vi "Assert Greater Or Equal_Variant.vi"(4 "Execution time (s)":dbl=-1.0, 5 "Assert Only? (F)":bool, 6 "error code (1)":i32=1, 7 "Label":string, 8 "error in (no error)":errorcluster, 9 "Register with caller test (F)":bool, 10 "Y":variant, 11 "X":variant) -> (0 "error out":errorcluster, 2 "Properties.Assert":refnum<class "Properties.Assert.lvclass">)   [LabVIEW 2020, in "Caraya.lvlib" / "Assert.lvclass"]
doc: "Generates an error if the input condition is not met.\n\n--\nCopyright © 2015 JKI All rights reserved.\n\nAuthor: Tomi Maila <tomi.maila@jki.net>\n\nThis library is provided \"AS IS\" ,WITHOUT WARRANTIES OR\nCONDITIONS OF ANY KIND, either express or implied.\n\nJKI -- jki.net"
uses:
  Assert.lvclass
  Assert.lvclass/Assert.ctl
  <userlib>/_OpenG.lib/string/string.llb/openg_string.lvlib
  Properties/Properties.lvclass
  Properties.Assert/Properties.Assert.lvclass
  C:/Projects/caraya/src/classes/Properties/Properties.lvclass
  C:/Projects/caraya/src/classes/Properties.Assert/Properties.Assert.lvclass
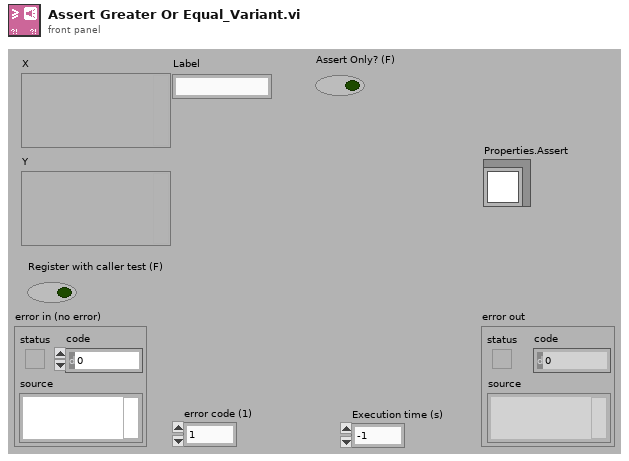
[diagram p1: front panel]
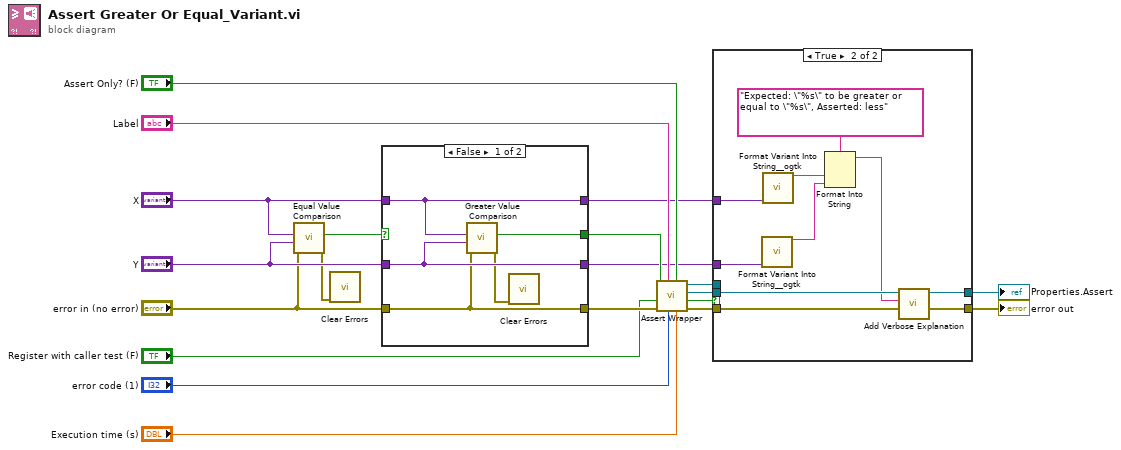
[diagram p0: block diagram]
diagram:
  n1 = call "Equal Value Comparison.vi"("error in (no error)"="error in (no error)", "Actual"="Y", "Expected"="X") -> ("error out"=w5:errorcluster, "Equal Values?"=w7:bool)  [unwired: 6 in, 1 out]
  n2 = call <vilib>:"Clear Errors.vi"("error in (no error)"=w5) -> ()  [unwired: 5 in, 2 out]
  n3 = case shown="False" w7 {
    selector: w7 -> [_ w28]
    tunnel: "X" -> [w25 w29]
    tunnel: [w25 w29] -> w13
    tunnel: [w23 w28] -> w12
    tunnel: "Y" -> [w24 w27]
    tunnel: [w24 w27] -> w11
    tunnel: "error in (no error)" -> [w22 w26]
    tunnel: [w22 w26] -> w10
    frame False {
      n4 = call "Greater Value Comparison.vi"("error in (no error)"=w22, "Y"=w24, "X"=w25) -> ("error out"=w21:errorcluster, "Asserted?"=w23:bool)  [unwired: 6 in, 1 out]
      n5 = call <vilib>:"Clear Errors.vi"("error in (no error)"=w21) -> ()  [unwired: 5 in, 2 out]
    }
    frame True {
    }
  }
  n6 = call "Assert Wrapper.vi"("Execution time (s)"="Execution time (s)", "Assert Only? (F)"="Assert Only? (F)", "error code (1)"="error code (1)", "Label"="Label", "error in (no error)"=w10, "Register with caller test (F)"="Register with caller test (F)", "Assert?"=w12) -> ("error out"=w16:errorcluster, "Verbose"=w14:bool, "Properties.Assert"=w2:refnum<class "Properties.Assert.lvclass">, "Assert out"=w3:refnum<class "Assert.lvclass">)  [unwired: 1 in]
  n7 = case shown="True" w14 {
    tunnel: [w31 w33] -> w15
    tunnel: w3 -> [_ _]
    tunnel: w16 -> [w31 w34]
    tunnel: w13 -> [_ w41]
    tunnel: w11 -> [_ w37]
    tunnel: w2 -> [w30 w36]
    tunnel: [w30 w32] -> w1
    frame False {
    }
    frame True {
      n8 = call <userlib>:"Format Variant Into String__ogtk.vi"("Variant"=w37) -> ("Output String"=w38:string)  [unwired: 13 in, 1 out]
      n9 = call <userlib>:"Format Variant Into String__ogtk.vi"("Variant"=w41) -> ("Output String"=w39:string)  [unwired: 13 in, 1 out]
      n10 = Format Into String(format string="Expected: \"%s\" to be greater or equal to \"%s\", Asserted: less" ("t"), w39, w38) -> (resulting string=w35:string)  [unwired: 2 in, 1 out]
      n11 = call "Add Verbose Explanation.vi"("error in (no error)"=w34, "Verbose Explanation"=w35, "Properties"=w36) -> ("error out"=w33:errorcluster, "Properties"=w32:refnum<class "Properties.Assert.lvclass">)  [unwired: 7 in]
    }
  }
  "error out" <- w15
  "Properties.Assert" <- w1
